vi "Event Record.vi"(8 "error in (no error)":errorcluster, 10 "Stream":refnum<class "Stream.lvclass">, 11 "Event in":refnum<class "Event.lvclass">) -> (0 "error out":errorcluster, 3 "Event out":refnum<class "Event.lvclass">)   [LabVIEW 2020, in "OpenLvVision_OpenCv.lvlib" / "Cuda.lvlib" / "Event.lvclass"]
doc: "Drops the event checkpoint into the specified CUDA stream."
uses:
  Event.lvclass
  C:/Users/lukas/Downloads/OpenLvVision_OpenCv/SourceCode/LabView/OpenLvVision_OpenCv/_LvHelpers/EdvrObject/EdvrObject.lvclass
  Stream/Stream.lvclass
  _LvHelpers/EdvrObject/EdvrObject.lvclass/EdvrObject.ctl
  OpenLvVision_OpenCv.lvlib
  _LvHelpers/EdvrObject/EdvrObject.lvclass
  <vilib>/Utility/error.llb/Error Cluster From Error Code.vi
  <vilib>/ErrorRing/Error Ring.xnode
  Dlls/OlvOpenCvWrapper.dll
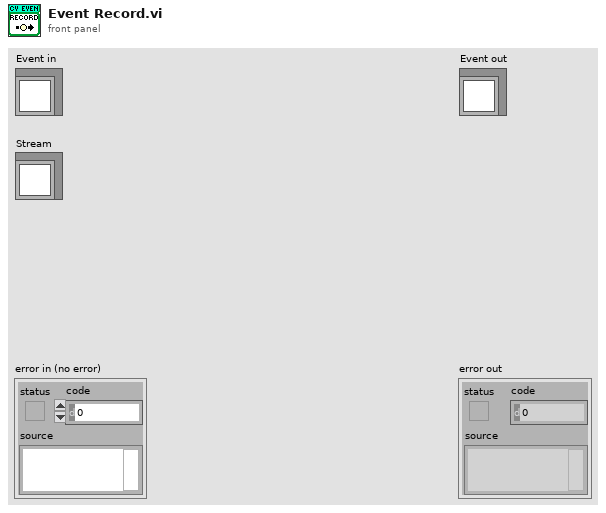
[diagram p1: front panel]
types:
  T1 = typedef "OpenLvVision_OpenCv.lvlib/EdvrObject.lvclass/Edvr.ctl" = refnum<data-value>
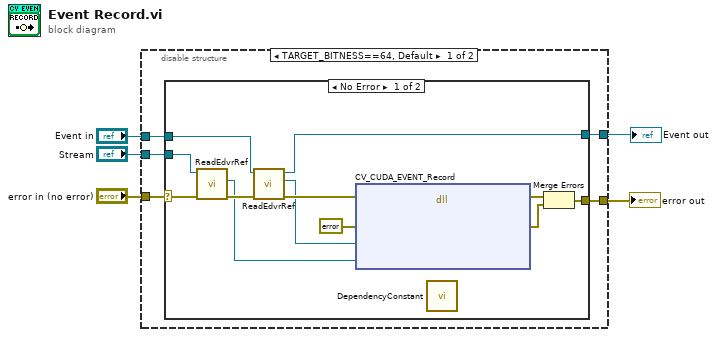
[diagram p0: block diagram]
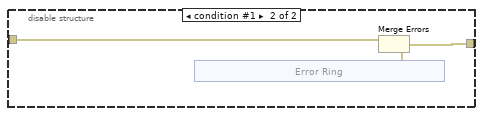
[diagram p3: hidden frame]
diagram:
  n1 = disable-structure shown="TARGET_BITNESS==64, Default" {
    disable-tunnel: "error in (no error)" -> [w6 w26]
    disable-tunnel: [w10 w27] -> w5
    disable-tunnel: [w9 _] -> w4
    disable-tunnel: "Event in" -> [w8 _]
    disable-tunnel: "Stream" -> [w7 _]
    frame condition #0 (active) {
      n2 = case shown="No Error" w6 {
        selector: w6 -> [w13 w24]
        tunnel: [w16 w24] -> w10
        tunnel: [w17 w23] -> w9
        tunnel: w8 -> [w15 w23]
        tunnel: w7 -> [w12 _]
        frame No Error {
          n3 = call "ReadEdvrRef.vi"("error in (no error)"=w13, "EdvrObject in"=w12) -> ("error out"=w14:errorcluster, "Edvr"=w11:T1)  [unwired: 7 in, 1 out]
          n4 = call "ReadEdvrRef.vi"("error in (no error)"=w14, "EdvrObject in"=w15) -> ("error out"=w19:errorcluster, "Edvr"=w18:T1, "EdvrObject out"=w17:refnum<class "Event.lvclass">)  [unwired: 7 in]
          n5 = dll-call lib="C:/Users/lukas/Downloads/OpenLvVision_OpenCv/SourceCode/LabView/OpenLvVision_OpenCv/Dlls/OlvOpenCvWrapper.dll" fn="CV_CUDA_EVENT_Record"(error in=w19, "Error"=errorcluster {"status"=FALSE, "code"=0, "source"=""} ("error out"), "eventEdvrRef"=w18, "streamEdvrRef"=w11) -> (error out=w22:errorcluster, "Error"=w21:errorcluster)  [unwired: 5 in, 1 out]
          n6 = call "DependencyConstant.vi"() -> ()  [unwired: 12 in]
          n7 = Merge Errors(w22, w21) -> (w16:errorcluster)
        }
        frame Error {
        }
      }
    }
    frame condition #1 {
      n8 = xnode "Error Ring"() -> ("error out"=w25:errorcluster)
      n9 = Merge Errors(w26, w25) -> (w27:errorcluster)
    }
  }
  "error out" <- w5
  "Event out" <- w4
